vi "MQTT Connect - Handle CONNACK properties.vi"(0 "MQTT session":T1, 5 "MQTT CONNACK Properties":T2[](array[typedef]) {"Property" items=["Payload Format Indicator"=1, "Message Expiry Interval"=2, "Content Type"=3, "Response Topic"=8, "Correlation Data"=9, "Subscription Identifier"=11, "Session Expiry Interval"=17, "Assigned Client Identifier"=18, "Server Keep Alive"=19, "Authentication Method"=21, "Authentication Data"=22, "Request Problem Information"=23, "Will Delay Interval"=24, "Request Response Information"=25, "Response Information"=26, "Server Reference"=28, "Reason String"=31, "Receive Maximum"=33, "Topic Alias Maximum"=34, "Topic Alias"=35, "Maximum QoS"=36, "Retain Available"=37, "User Property"=38, "Maximum Packet Size"=39, "Wildcard Subscription Available"=40, "Subscription Identifier Available"=41, "Shared Subscription Available"=42]}, 11 "error in (no error)":errorcluster) -> (4 "MQTT session out":T1, 15 "error out":errorcluster)   [LabVIEW 2019, in "KoRE-MQTT.lvlib"]
doc: "Copyright (c) 2026 KoRElibs.com\nSPDX-License-Identifier: EUPL-1.2\n\nThis VI is licensed under the European Union Public License (EUPL) Version 1.2. You may use this VI unmodified in proprietary works. If you distribute a modified version of this file, the modified file must be released under the EUPL-1.2. Full license: https://joinup.ec.europa.eu/asset/eupl/eupl/1.2/\n\nCopyright (c) 2025 KoRElibs.com\nSPDX-License-Identifier: EUPL-1.2\n\nThis VI is licensed under the European Union Public License (EUPL) Version 1.2. You may use this VI unmodified in proprietary works. If you distribute a modified version of this file, the modified file must be released under the EUPL-1.2. Full license: https://joinup.ec.europa.eu/asset/eupl/eupl/1.2/"
uses:
  KoRE-MQTT.lvlib
  Public/TypeDefs/MQTT Client Session.ctl
  Public/TypeDefs/MQTT Property - GENERIC.ctl
  Public/TypeDefs/MQTT Property Type.ctl
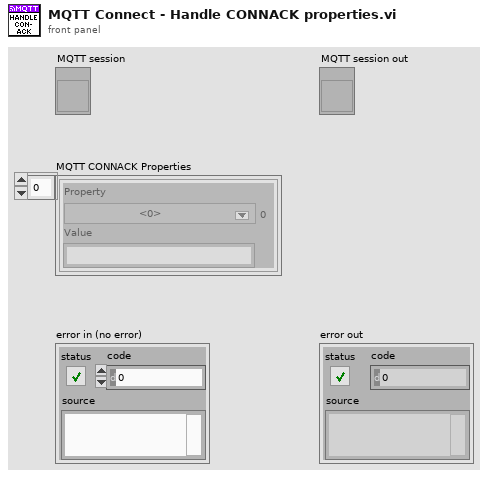
[diagram p1: front panel]
types:
  T1 = typedef "KoRE-MQTT.lvlib/MQTT Client Session.ctl" = refnum<vi>
  T2 = typedef "KoRE-MQTT.lvlib/MQTT Property - GENERIC.ctl" = cluster{"Property":T3, "Value":string}
  T3 = typedef "KoRE-MQTT.lvlib/MQTT Property Type.ctl" = u8
  T4 = typedef "KoRE-MQTT.lvlib/MQTT Client Session - Data.ctl" = cluster{"TCP ref":refnum<k5>, "Next Packet Id":u16, "Version":u8, "Host":string, "Port":u16, "Ping Delta":u32, "Username":string, "Password":string, "Will QoS":u8, "Will Retain":bool, "Will Topic":string, "Will Payload":string, "TCP Timeout":i32, "Semaphore":T5, "In-Flight Messages":variant, "Close":bool, "Last Send":u32, "Keep Alive":u16, "Last Ping RTT":u32, "Last Ping":u32, "Will Properties":T6[], "Session Expiry Interval":u32, "Maximum QoS":u8, "Retain Available":bool, "Server Maximum Packet Size":u32, "Client Identifier":string, "Server Topic Alias Maximum":u16, "Wildcard Subscription Available":bool, "Subscription Identifier Available":bool, "Shared Subscription Available":bool, "Connect Properties":T7[], "Client Maximum Packet Size":u32, "Client Topic Alias Maximum":u16, "Server Receive Maximum":u16, "Client Receive Maximum":u16, "TLS cfg":refnum<k36>, "Subscriptions":T8[]}
  T5 = typedef "Semaphore RefNum" = refnum<k1>
  T6 = typedef "KoRE-MQTT.lvlib/MQTT Property - Will.ctl" = cluster{"Property":u8, "Value":string}
  T7 = typedef "KoRE-MQTT.lvlib/MQTT Property - CONNECT.ctl" = cluster{"Property":u8, "Value":string}
  T8 = typedef "KoRE-MQTT.lvlib/MQTT Subscription - Info.ctl" = cluster{"Packet Id":u16, "Index":u16, "Identifier":u32, "QoS":u8, "Topic Filter":string, "Reason Code":u8, "Reason String":string, "Granted":bool}
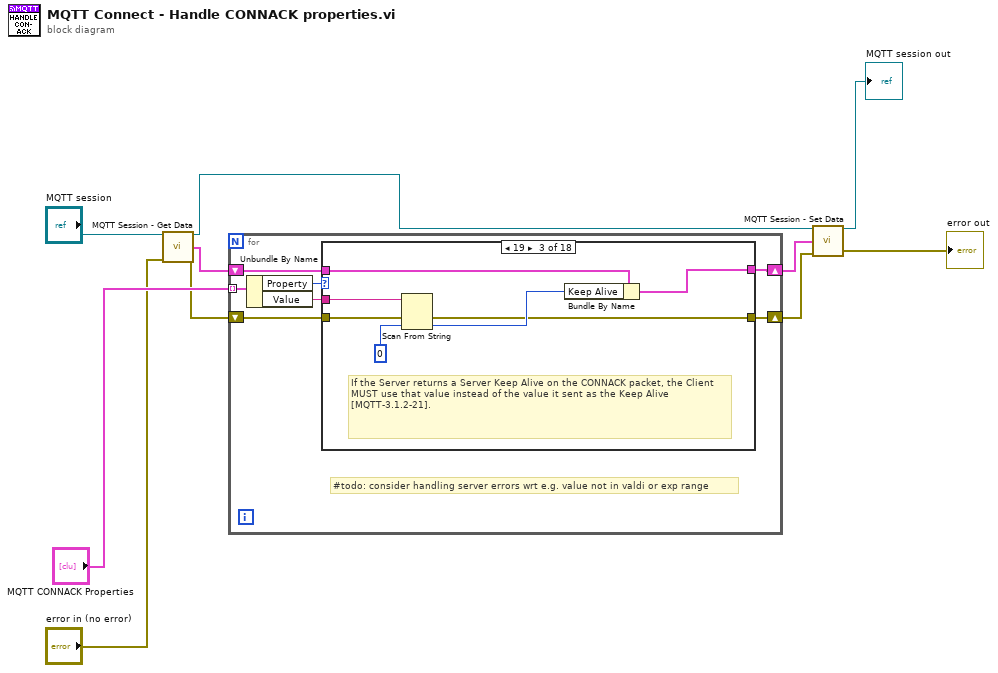
[diagram p0: block diagram]
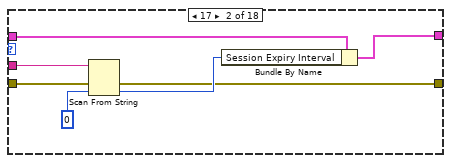
[diagram p3: hidden frame]
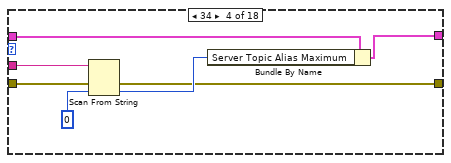
[diagram p4: hidden frame]
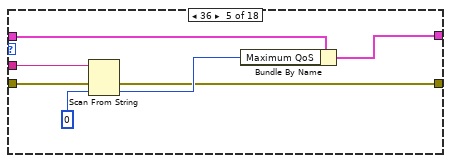
[diagram p5: hidden frame]
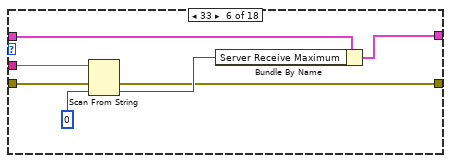
[diagram p6: hidden frame]
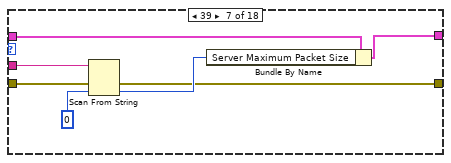
[diagram p7: hidden frame]
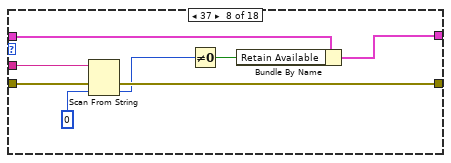
[diagram p8: hidden frame]
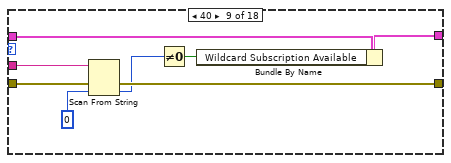
[diagram p9: hidden frame]
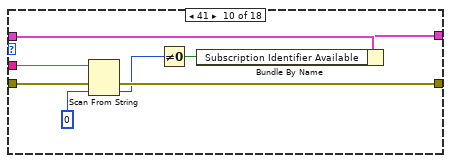
[diagram p10: hidden frame]
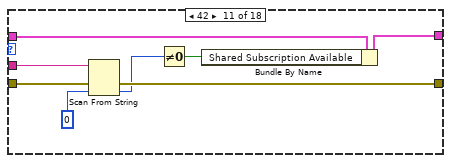
[diagram p11: hidden frame]
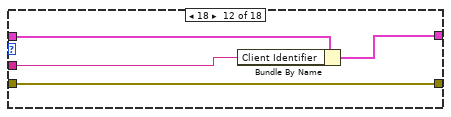
[diagram p12: hidden frame]
diagram:
  n1 = call "MQTT Session - Get Data.vi"("mqtt ref in"="MQTT session", "error in"="error in (no error)") -> ("mqtt ref out"=w6:T1, "mqtt ref data"=w5:T4, "error out"=w1:errorcluster)  [unwired: 11 in]
  n2 = for {
    tunnel: "MQTT CONNACK Properties" -> [w17] mode=indexing
    shift-right: [w13] -> w8
    shift-left: w5 -> [w15]
    shift-right: [w12] -> w7
    shift-left: w1 -> [w11]
    # "#todo: consider handling server errors wrt e.g. value not in valdi or exp range"
    n3 = Unbundle By Name(w17) -> ("Property"=w16:T3, "Value"=w14:string)
    n4 = case shown="19" w16 {
      tunnel: w15 -> [w19 w26 w33 w40 w47 w54 w61 w69 w77 w85 w93 w97 w99 w101 w103 w105 w107 w109]
      tunnel: w14 -> [_ w24 w31 w38 w45 w52 w59 w67 w75 w83 w91 w95 _ _ _ _ _ _]
      tunnel: [w19 w22 w29 w36 w43 w50 w57 w66 w74 w82 w90 w96 w99 w101 w103 w105 w107 w109] -> w13
      tunnel: [w18 w21 w28 w35 w42 w49 w56 w65 w73 w81 w89 w94 w98 w100 w102 w104 w106 w108] -> w12
      tunnel: w11 -> [w18 w20 w27 w34 w41 w48 w55 w64 w72 w80 w88 w94 w98 w100 w102 w104 w106 w108]
      frame Default {
        # "#todo: ERROR unexpected Property,"
      }
      frame 17 {
        n5 = Scan From String(input string=w24, error in=w20, default 1=u32 0 ("Session Expiry Interval")) -> (error out=w21:errorcluster, output 1=w23:u32)  [unwired: 2 in, 2 out]
        n6 = Bundle By Name(cluster=w26, "Session Expiry Interval"=w23) -> (w22:T4)
      }
      frame 19 {
        # "If the Server returns a Server Keep Alive on the CONNACK packet, the Client MUST use that value instead of the value it sent as the Keep Alive [MQTT-3.1.2-21]."
        n7 = Scan From String(input string=w31, error in=w27, default 1=u16 0 ("Session Expiry Interval")) -> (error out=w28:errorcluster, output 1=w30:u16)  [unwired: 2 in, 2 out]
        n8 = Bundle By Name(cluster=w33, "Keep Alive"=w30) -> (w29:T4)
      }
      frame 34 {
        n9 = Scan From String(input string=w38, error in=w34, default 1=u16 0 ("Session Expiry Interval")) -> (error out=w35:errorcluster, output 1=w37:u16)  [unwired: 2 in, 2 out]
        n10 = Bundle By Name(cluster=w40, "Server Topic Alias Maximum"=w37) -> (w36:T4)
      }
      frame 36 {
        n11 = Scan From String(input string=w45, error in=w41, default 1=u8 0 ("Session Expiry Interval")) -> (error out=w42:errorcluster, output 1=w44:u8)  [unwired: 2 in, 2 out]
        n12 = Bundle By Name(cluster=w47, "Maximum QoS"=w44) -> (w43:T4)
      }
      frame 33 {
        n13 = Scan From String(input string=w52, error in=w48, default 1=u16 0 ("Session Expiry Interval")) -> (error out=w49:errorcluster, output 1=w51:u16)  [unwired: 2 in, 2 out]
        n14 = Bundle By Name(cluster=w54, "Server Receive Maximum"=w51) -> (w50:T4)
      }
      frame 39 {
        n15 = Scan From String(input string=w59, error in=w55, default 1=u32 0 ("Session Expiry Interval")) -> (error out=w56:errorcluster, output 1=w58:u32)  [unwired: 2 in, 2 out]
        n16 = Bundle By Name(cluster=w61, "Server Maximum Packet Size"=w58) -> (w57:T4)
      }
      frame 37 {
        n17 = Scan From String(input string=w67, error in=w64, default 1=u8 0 ("Session Expiry Interval")) -> (error out=w65:errorcluster, output 1=w63:u8)  [unwired: 2 in, 2 out]
        n18 = Not Equal To 0?(x=w63) -> (x != 0?=w62:bool)
        n19 = Bundle By Name(cluster=w69, "Retain Available"=w62) -> (w66:T4)
      }
      frame 40 {
        n20 = Scan From String(input string=w75, error in=w72, default 1=u8 0 ("Session Expiry Interval")) -> (error out=w73:errorcluster, output 1=w71:u8)  [unwired: 2 in, 2 out]
        n21 = Not Equal To 0?(x=w71) -> (x != 0?=w70:bool)
        n22 = Bundle By Name(cluster=w77, "Wildcard Subscription Available"=w70) -> (w74:T4)
      }
      frame 41 {
        n23 = Scan From String(input string=w83, error in=w80, default 1=u8 0 ("Session Expiry Interval")) -> (error out=w81:errorcluster, output 1=w79:u8)  [unwired: 2 in, 2 out]
        n24 = Not Equal To 0?(x=w79) -> (x != 0?=w78:bool)
        n25 = Bundle By Name(cluster=w85, "Subscription Identifier Available"=w78) -> (w82:T4)
      }
      frame 42 {
        n26 = Scan From String(input string=w91, error in=w88, default 1=u8 0 ("Session Expiry Interval")) -> (error out=w89:errorcluster, output 1=w87:u8)  [unwired: 2 in, 2 out]
        n27 = Not Equal To 0?(x=w87) -> (x != 0?=w86:bool)
        n28 = Bundle By Name(cluster=w93, "Shared Subscription Available"=w86) -> (w90:T4)
      }
      frame 18 {
        n29 = Bundle By Name(cluster=w97, "Client Identifier"=w95) -> (w96:T4)
      }
      frame 21 {
        # "Authentication Method"
      }
      frame 22 {
        # "Authentication Data"
      }
      frame 26 {
        # "Response Information"
      }
      frame 28 {
        # "Server Reference"
      }
      frame 31 {
        # "Reason String"
      }
      frame 38 {
        # "User Property"
      }
    }
  }
  n30 = call "MQTT Session - Set Data.vi"("mqtt ref in"=w6, "mqtt ref data"=w8, "error in"=w7) -> ("mqtt ref out"=→"MQTT session out":T1, "error out"=→"error out":errorcluster)  [unwired: 11 in]
